vi "Add Extensions to Web Service.vi"(8 "error in (no error)":errorcluster, 11 "Project":path=path "P:/alsmith/Sales/users/ACS/LabVIEW Continuous Integration/Core/LabVIEW CI Service/LabVIEW CI Service.lvproj") -> (0 "error out":errorcluster)   [LabVIEW 2014]
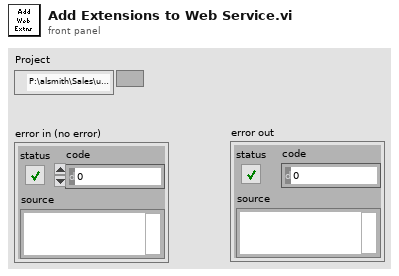
[diagram p1: front panel]
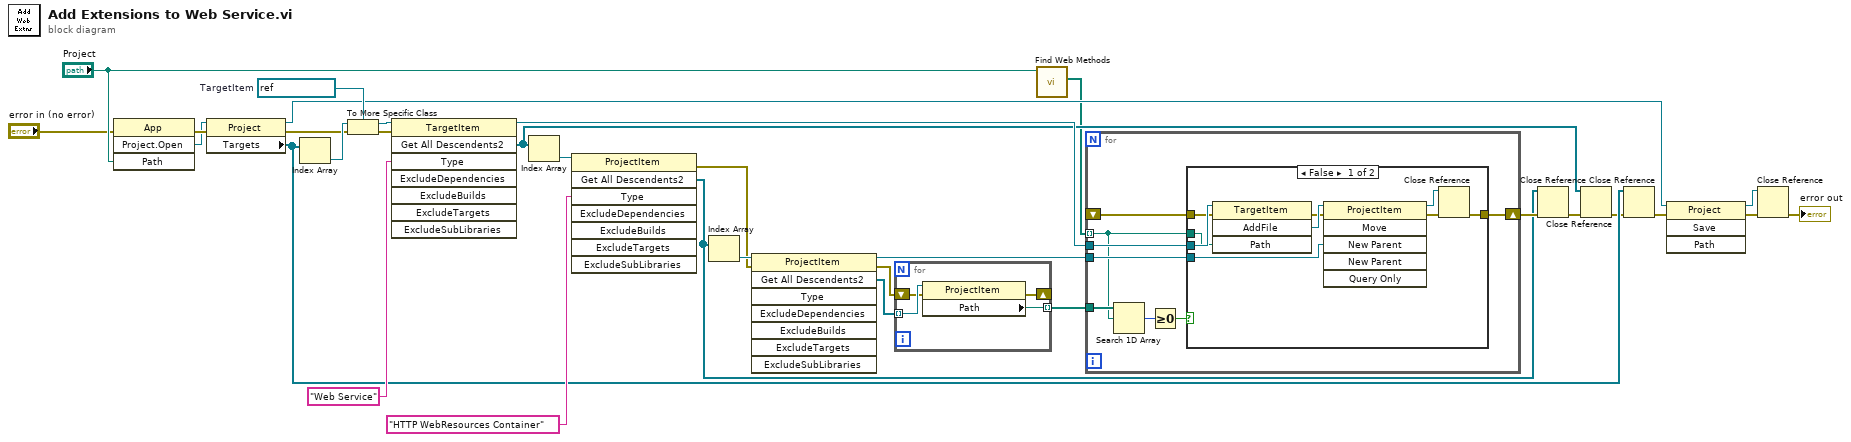
[diagram p0: block diagram]
diagram:
  w31 = refnum<vi> refnum  # TargetItem
  n1 = invoke class="App" method="Project.Open"(error in="error in (no error)", "Path"="Project") -> (error out=w29:errorcluster, "Project:Open"=w25:refnum<vi>)  [unwired: 2 in, 2 out]
  n2 = property class="Project"(reference=w25, error in=w29) -> (reference out=w22:refnum<vi>, error out=w28:errorcluster, "Targets"=w12:refnum<vi>[])
  n3 = Index Array(array=w12) -> (element=w30:refnum<vi>)  [unwired: 1 in]
  n4 = To More Specific Class(target class=w31, reference=w30, error in=w28) -> (specific class reference=w24:refnum<vi>, error out=w27:errorcluster)
  n5 = invoke class="TargetItem" method="Get All Descendents2"(reference=w24, error in=w27, "Type"="Web Service") -> (reference out=w19:refnum<vi>, "Get All Descendents2"=w13:refnum<vi>[])  [unwired: 5 in, 6 out]
  n6 = Index Array(array=w13) -> (element=w21:refnum<vi>)  [unwired: 1 in]
  n7 = invoke class="ProjectItem" method="Get All Descendents2"(reference=w21, "Type"="HTTP WebResources Container" ("Type String")) -> (error out=w4:errorcluster, "Get All Descendents2"=w14:refnum<vi>[])  [unwired: 6 in, 6 out]
  n8 = Index Array(array=w14) -> (element=w6:refnum<vi>)  [unwired: 1 in]
  n9 = invoke class="ProjectItem" method="Get All Descendents2"(reference=w6, error in=w4) -> (reference out=w5:refnum<vi>, error out=w1:errorcluster, "Get All Descendents2"=w3:refnum<vi>[])  [unwired: 6 in, 5 out]
  n10 = for {
    tunnel: w3 -> [w35] mode=indexing
    tunnel: [w34] -> w2 mode=indexing
    shift-right: [w32] -> _
    shift-left: w1 -> [w33]
    n11 = property class="ProjectItem"(reference=w35, error in=w33) -> (error out=w32:errorcluster, "Path"=w34:path)  [unwired: 1 out]
  }
  n12 = call "Find Web Methods.vi"("Project"="Project") -> ("Web Methods"=w10:path[])  [unwired: 10 in]
  n13 = for {
    tunnel: w19 -> [w43]
    tunnel: w5 -> [w41]
    shift-right: [w36] -> w16
    shift-left: _ -> [w42]
    tunnel: w10 -> [w39] mode=indexing
    tunnel: w2 -> [w40]
    n14 = Search 1D Array(1D array=w40, element=w39) -> (index of element=w38:i32)  [unwired: 1 in]
    n15 = Greater Or Equal To 0?(x=w38) -> (x >= 0?=w37:bool)
    n16 = case shown="False" w37 {
      tunnel: w43 -> [w52 _]
      tunnel: w42 -> [w51 w53]
      tunnel: [w44 w53] -> w36
      tunnel: w41 -> [w49 _]
      tunnel: w39 -> [w47 _]
      frame False {
        n17 = invoke class="TargetItem" method="AddFile"(reference=w52, error in=w51, "Path"=w47) -> (error out=w48:errorcluster, "AddFile"=w50:refnum<vi>)  [unwired: 1 in, 2 out]
        n18 = invoke class="ProjectItem" method="Move"(reference=w50, error in=w48, "New Parent"=w49) -> (reference out=w46:refnum<vi>, error out=w45:errorcluster)  [unwired: 3 in, 4 out]
        n19 = Close Reference(reference=w46, error in (no error)=w45) -> (error out=w44:errorcluster)
      }
      frame True {
      }
    }
  }
  n20 = Close Reference(reference=w14, error in (no error)=w16) -> (error out=w15:errorcluster)
  n21 = Close Reference(reference=w13, error in (no error)=w15) -> (error out=w9:errorcluster)
  n22 = Close Reference(reference=w12, error in (no error)=w9) -> (error out=w8:errorcluster)
  n23 = invoke class="Project" method="Save"(reference=w22, error in=w8) -> (reference out=w17:refnum<vi>, error out=w20:errorcluster)  [unwired: 2 in, 2 out]
  n24 = Close Reference(reference=w17, error in (no error)=w20) -> (error out=→"error out":errorcluster)
